vi "Main - Add Local Chassis.vi"(8 "error in (no error)":errorcluster, 11 "Node Ptr":u64 format="%.0x") -> (0 "error out":errorcluster)   [LabVIEW 2020, in "SEECD System Explorer.lvlib"]
uses:
  SEECD System Explorer.lvlib
  Shared/Type Defs/Local Chassis Settings.ctl
  Scripting/Scan Engine Scripting.lvlib
  Shared/SEECD Shared.lvlib
panel:
  in  "Tag":string
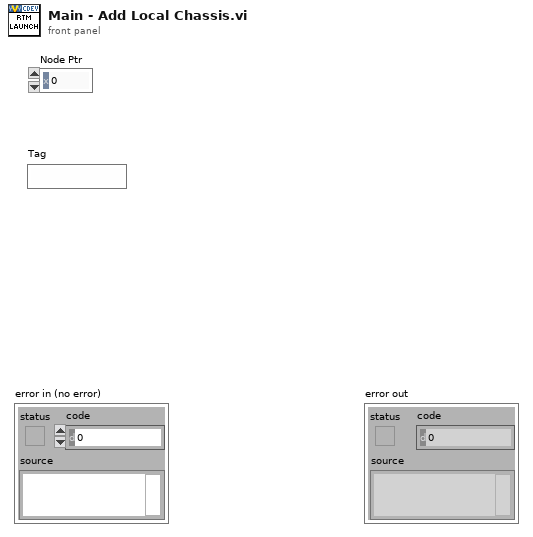
[diagram p1: front panel]
types:
  T1 = typedef "SEECD Shared.lvlib/Local Chassis Settings.ctl" = cluster{"name":string, "number of slots":i32}
  T2 = typedef "Custom Device API.lvlib/Custom Device Item Ref.ctl" = u64
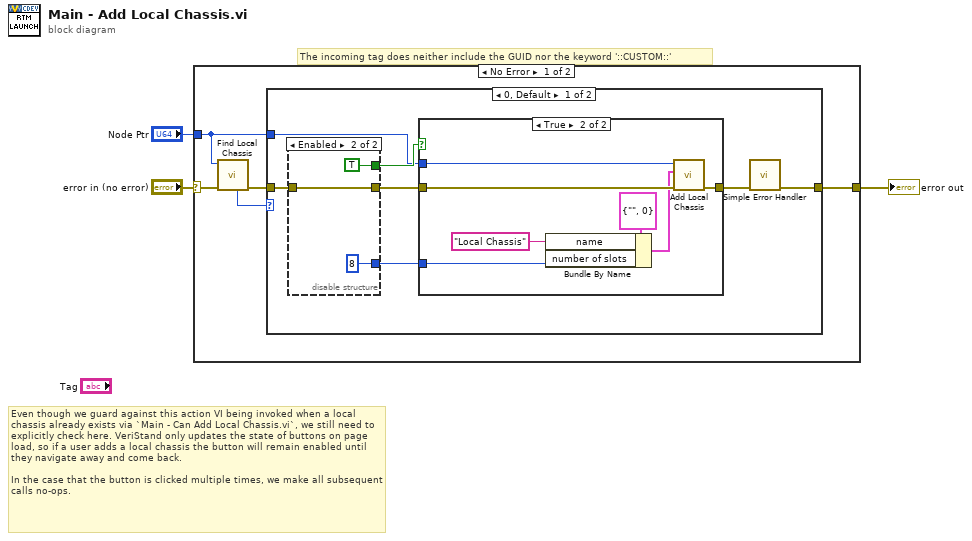
[diagram p0: block diagram]
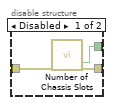
[diagram p2: hidden frame]
diagram:
  # "Even though we guard against this action VI being invoked when a local chassis already exists via `Main - Can Add Local Chassis.vi`, we still need to explicitly check here. VeriStand only updates the state of buttons on page load, so if a user adds a local chassis the button will remain enabled until they navigate away and come back.\n\nIn the case that the button is clicked multiple times, we make all subsequent calls no-ops."
  # "The incoming tag does neither include the GUID nor the keyword '::CUSTOM::'"
  n1 = case shown="No Error" "error in (no error)" {
    selector: "error in (no error)" -> [w7 w31]
    tunnel: "Node Ptr" -> [w5 _]
    tunnel: [w8 w31] -> w1
    frame No Error {
      n2 = call "Find Local Chassis.vi"("error in"=w7, "scan engine custom device ref in"=w5) -> ("error out"=w6:errorcluster, "user variables ref"=w4:T2)  [unwired: 4 in, 4 out]
      n3 = case shown="0, Default" w4 {
        tunnel: [w9 w30] -> w8
        tunnel: w6 -> [w12 w30]
        tunnel: w5 -> [w11 _]
        frame 0, Default {
          n4 = disable-structure shown="Enabled" {
            disable-tunnel: [_ 8 ("# Slots")] -> w15
            disable-tunnel: [w18 w19] -> w14
            disable-tunnel: [w17 TRUE ("OK")] -> w13
            disable-tunnel: w12 -> [w16 w19]
            frame Disabled {
              n5 = call "Number of Chassis Slots"("error in (no error)"=w16) -> ("OK"=w17:bool, "error out"=w18:errorcluster)  [unwired: 16 in, 1 out]
            }
            frame Enabled {
            }
          }
          n6 = case shown="True" w13 {
            tunnel: w15 -> [_ w24]
            tunnel: w11 -> [_ w29]
            tunnel: w14 -> [w22 w28]
            tunnel: [w22 w27] -> w10
            frame False {
            }
            frame True {
              n7 = Bundle By Name(cluster=T1 {"name"="", "number of slots"=0} ("settings"), "name"="Local Chassis" ("Section Name"), "number of slots"=w24) -> (w23:T1)
              n8 = call "Add Local Chassis.vi"("error in"=w28, "settings"=w23, "scan engine custom device ref in"=w29) -> ("error out"=w27:errorcluster)  [unwired: 4 in, 4 out]
            }
          }
          n9 = call <vilib>:"Simple Error Handler.vi"("error in (no error)"=w10) -> ("error out"=w9:errorcluster)  [unwired: 4 in, 4 out]
        }
        frame 1 {
        }
      }
    }
    frame Error {
    }
  }
  "error out" <- w1
